vi "File Integrity Guard.vi"(8 "error in":errorcluster, 11 "File Path":path) -> (0 "error out":errorcluster)   [LabVIEW 2026]
doc: "This VI checks the hash value of the provided file against the hash whitelist constant. If the file is not authorized an error is produced."
uses:
  <vilib>/security/Message Digest/API/Instances/File/SHA-512 File Checksum.vi
  <vilib>/security/Message Digest/API/NI_Message Digest API.lvlib
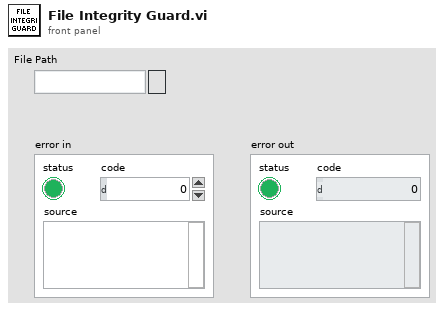
[diagram p1: front panel]
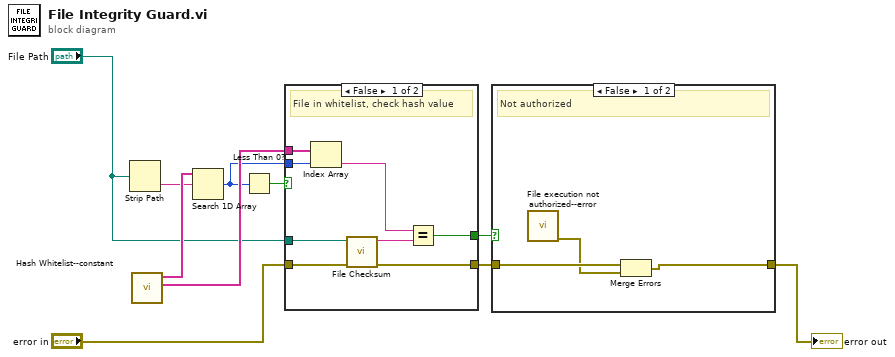
[diagram p0: block diagram]
diagram:
  n1 = Strip Path(path="File Path") -> (name=w6:string)  [unwired: 1 out]
  n2 = call "Hash Whitelist--constant.vi"() -> ("Hash Values"=w4:string[], "Files"=w7:string[])  [unwired: 10 in]
  n3 = Search 1D Array(1D array=w7, element=w6) -> (index of element=w3:i32)  [unwired: 1 in]
  n4 = Less Than 0?(x=w3) -> (x < 0?=w5:bool)
  n5 = case shown="False" w5 {
    tunnel: w4 -> [w16 _]
    tunnel: w3 -> [w15 _]
    tunnel: "File Path" -> [w14 _]
    tunnel: "error in" -> [w18 w19]
    tunnel: [w11 _] -> w1
    tunnel: [w17 w19] -> w9
    frame False {
      # "File in whitelist, check hash value"
      n6 = Index Array(array=w16, index=w15) -> (element=w12:string)
      n7 = call-poly <vilib>:"File Checksum.vi"("error in"=w18, "path"=w14) -> ("error out"=w17:errorcluster, "digest"=w13:string)  [unwired: 8 in]
      n8 = Equal?(x=w12, y=w13) -> (x = y?=w11:bool)
    }
    frame True {
      # "File not found."
    }
  }
  n9 = case shown="False" w1 {
    tunnel: w9 -> [w22 w23]
    tunnel: [w20 w23] -> w8
    frame False {
      # "Not authorized"
      n10 = call "File execution not authorized--error.vi"() -> ("error out"=w21:errorcluster)  [unwired: 11 in]
      n11 = Merge Errors(w22, w21) -> (w20:errorcluster)
    }
    frame True {
      # "Authorized"
    }
  }
  "error out" <- w8
